vi "RemoteVI Demo Layout.vi"(0 "path":path, 11 "error in":errorcluster) -> (15 "error out":errorcluster)   [LabVIEW 2020]
doc: "Lays out the front panel of RemoteVI Demo.vi (the generator places a graph or chart far larger than the window and stacks the controls under it) and saves it: controls in a column on the left, the graph to their right, Ask with Answer and Open File with File in two rows below the graph with a 400 x 230 plot area, its graph palette (zoom, pan) visible and autoscaling off on both scales (Scale Fit 0, so a zoom is not undone by the next data write), the window sized to the content. Run it once after regenerating the demo, with the demo idle."
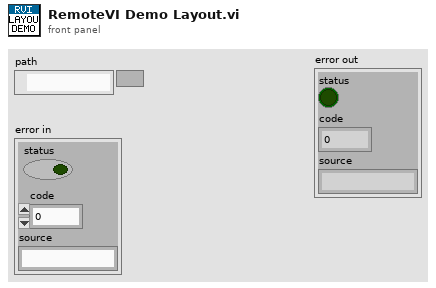
[diagram p1: front panel]
types:
  T1 = cluster{"Left":i32, "Top":i32, "Right":i32, "Bottom":i32}
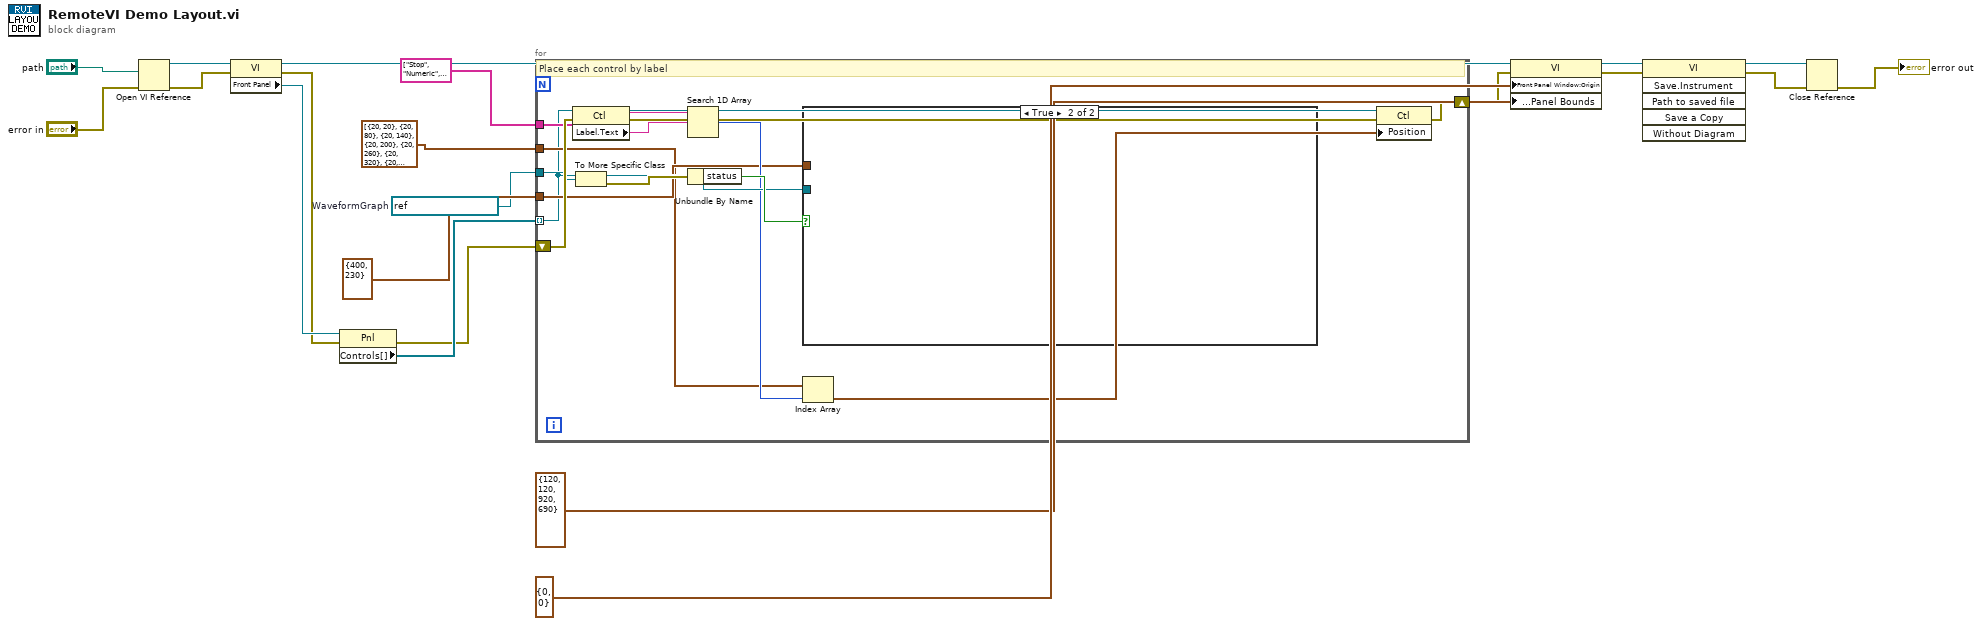
[diagram p0: block diagram]
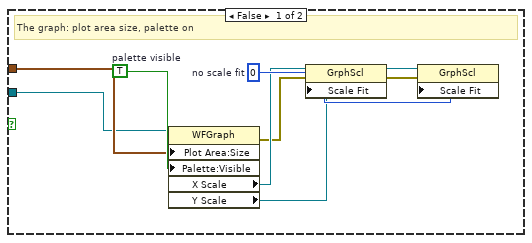
[diagram p2: hidden frame]
diagram:
  w12 = refnum<vi> refnum  # WaveformGraph
  n1 = Open VI Reference(vi path="path", error in (no error)="error in") -> (vi reference=w3:refnum<vi>, error out=w4:errorcluster)  [unwired: 4 in]
  n2 = property class="VI"(reference=w3, error in=w4) -> (reference out=w5:refnum<vi>, error out=w6:errorcluster, "Front Panel"=w7:refnum<vi>)
  n3 = property class="Pnl"(reference=w7, error in=w6) -> (error out=w8:errorcluster, "Controls[]"=w9:refnum<vi>[])  [unwired: 1 out]
  n4 = for {
    tunnel: string[] ["Stop", "Numeric", "Mode", "Enable", "Message", "URL", "error out", "Sine", "Ask", "Answer", "Open File", "File"] -> [w23]
    tunnel: cluster{"Left":i32, "Top":i32}[] [{"Left"=20, "Top"=20}, {"Left"=20, "Top"=80}, {"Left"=20, "Top"=140}, {"Left"=20, "Top"=200}, {"Left"=20, "Top"=260}, {"Left"=20, "Top"=320}, {"Left"=20, "Top"=380}, {"Left"=220, "Top"=20}, {"Left"=240, "Top"=385}, {"Left"=330, "Top"=388}, {"Left"=240, "Top"=440}, {"Left"=330, "Top"=443}] -> [w24]
    tunnel: w12 -> [w25]
    tunnel: cluster{"Width":i32, "Height":i32} {"Width"=400, "Height"=230} -> [w26]
    tunnel: w9 -> [w22] mode=indexing
    shift-right: [w28] -> w14
    shift-left: w8 -> [w27]
    # "Place each control by label"
    n5 = property class="Ctl"(reference=w22, error in=w27) -> (reference out=w29:refnum<vi>, error out=w30:errorcluster, "Label.Text"=w31:string)
    n6 = To More Specific Class(target class=w25, reference=w22) -> (specific class reference=w34:refnum<vi>, error out=w35:errorcluster)  [unwired: 1 in]
    n7 = Search 1D Array(1D array=w23, element=w31) -> (index of element=w32:i32)  [unwired: 1 in]
    n8 = Unbundle By Name(w35) -> ("status"=w36:bool)
    n9 = case shown="True" w36 {
      tunnel: w26 -> [w38 _]
      tunnel: w34 -> [w37 _]
      frame False {
        w43 = u8 0  # no scale fit
        w39 = TRUE  # palette visible
        # "The graph: plot area size, palette on"
        n10 = property class="WFGraph"(reference=w37, "Plot Area:Size"=w38, "Palette:Visible"=w39) -> (error out=w40:errorcluster, "X Scale"=w41:refnum<vi>, "Y Scale"=w42:refnum<vi>)  [unwired: 1 in, 1 out]
        n11 = property class="GrphScl"(reference=w41, error in=w40, "Scale Fit"=w43) -> (error out=w44:errorcluster)  [unwired: 1 out]
        n12 = property class="GrphScl"(reference=w42, error in=w44, "Scale Fit"=w43) -> ()  [unwired: 2 out]
      }
      frame True {
      }
    }
    n13 = Index Array(array=w24, index=w32) -> (element=w33:cluster{"Left":i32, "Top":i32})
    n14 = property class="Ctl"(reference=w29, error in=w30, "Position"=w33) -> (error out=w28:errorcluster)  [unwired: 1 out]
  }
  n15 = property class="VI"(reference=w5, error in=w14, "Front Panel Window:Origin"=cluster{"Horizontal":i32, "Vertical":i32} {"Horizontal"=0, "Vertical"=0}, "Front Panel Window:Panel Bounds"=T1 {"Left"=120, "Top"=120, "Right"=920, "Bottom"=690}) -> (reference out=w17:refnum<vi>, error out=w18:errorcluster)
  n16 = invoke class="VI" method="Save.Instrument"(reference=w17, error in=w18) -> (reference out=w19:refnum<vi>, error out=w20:errorcluster)  [unwired: 4 in, 4 out]
  n17 = Close Reference(reference=w19, error in (no error)=w20) -> (error out=→"error out":errorcluster)
